vi "LUX_Intensity_test.vi"(8 "error in (no error)":errorcluster) -> (0 "error out":errorcluster)   [LabVIEW 2025]
uses:
  SubVIs/All test cluster.ctl
  SubVIs/All_enum_ctl.ctl
  SubVIs/Arduino_lamps.ctl
  SubVIs/Lamps_global.vi
  <vilib>/Utility/file.llb/Write Delimited Spreadsheet (string).vi
  <instrlib>/BK Precision 9200 Series/BK Precision 9200 Series.lvlib
  <instrlib>/Keithley 2260B/Keithley 2260B.lvlib
panel:
  in  "ESP PORT":refnum<visa-resource-name>
  out "Connected? 2":bool caption="Long Blank Button"
  in  "LUX VALUE":dbl
  out "Status":string
  in  "POWER SUPPLY":bool caption="Blank Button"
  out "Text name":string
  in  "COM PORT:":refnum<visa-resource-name>
  in  "Start/Stop":bool caption="Slide Switch"
  in  "File Path:":path
  in  "FILENAME":string
  out "Table":string[][](table)
  out "Connected?":bool caption="Long Blank Button"
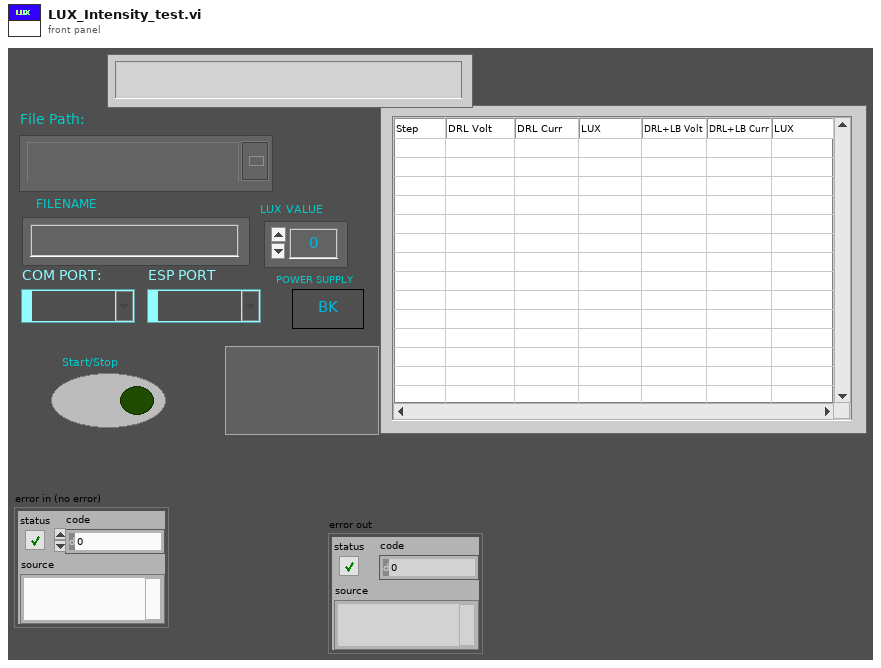
[diagram p1: front panel]
types:
  T1 = enum32{"Invalid", "Standard", "Closed", "Hidden", "Minimized", "Maximized"}
  T2 = typedef "All_enum_ctl.ctl" = enum16{"Init", "Poll", "Connect_esp32", "Connect", "check_start", "Start", "Set_Voltage", "On_relay", "Read_Voltage", "Off_Relay", "Next_Relay", "Next_Step", "Stop", "Store", "Error", "Exit"}
  T3 = typedef "All test cluster.ctl" = cluster{"FilePath":path, "Test Status":bool, "Start Volt":dbl, "End Volt":dbl, "Present Step":dbl, "Present Time(s)":dbl, "End Time":dbl, "Table":string[], "Intensity":string, "BK/Keith":bool, "COM":refnum<visa-resource-name>, "Next state":T2, "Step no.":dbl, "Start ms":u32, "ESP_COM":refnum<visa-resource-name>, "Relay_no":dbl, "Datas":string[]}
  T4 = typedef "Arduino_lamps.ctl" = enum16{"Init", "Poll", "Read", "Write", "Exit"}
  T5 = cluster{"Baud Rate":u32, "Parity":u16, "Data Bits":u16, "Stop Bits":u16, "Flow Control":u16}
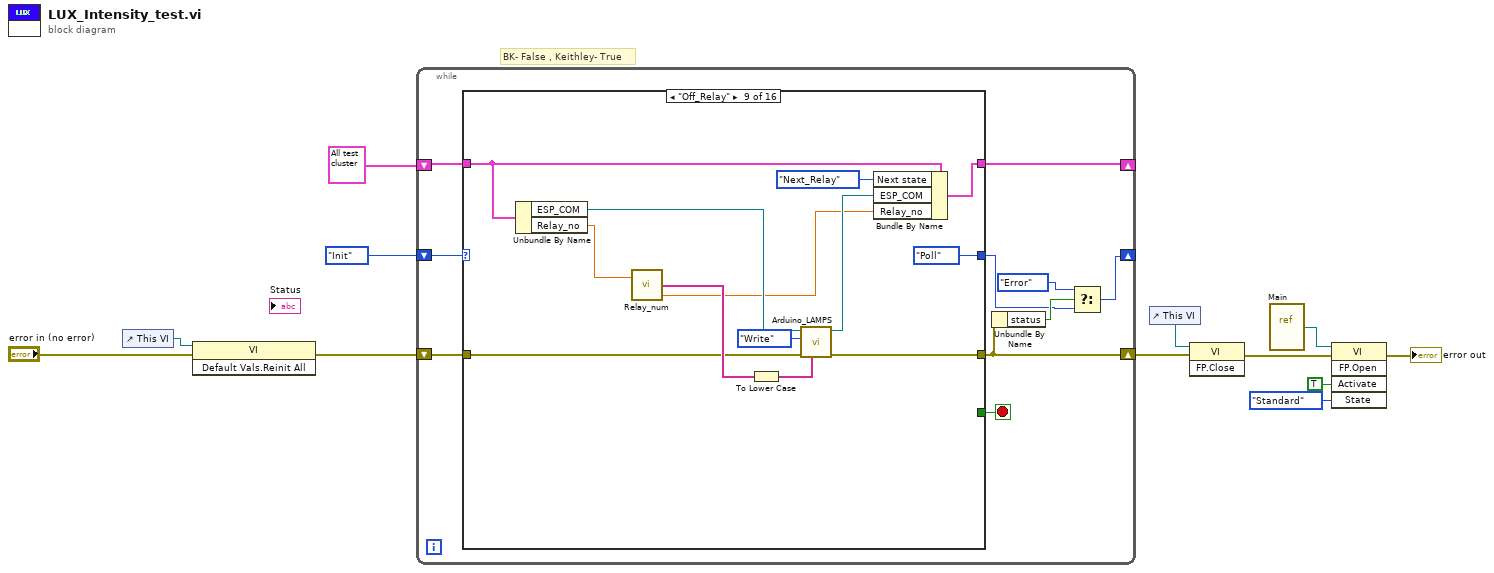
[diagram p0: block diagram]
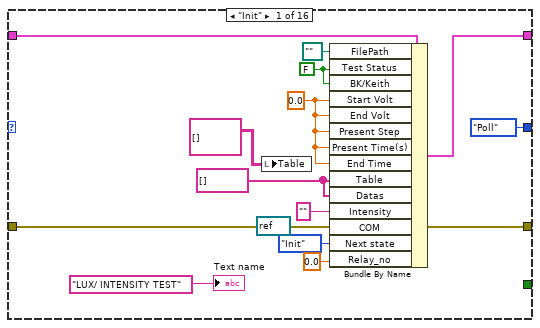
[diagram p2: hidden frame]
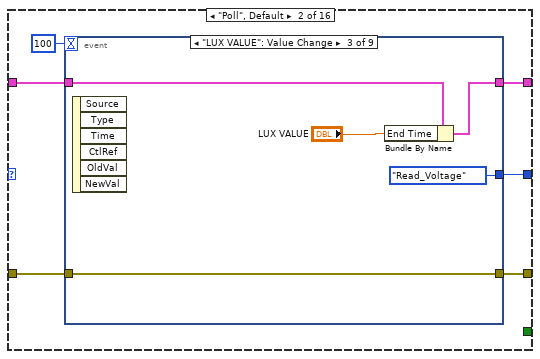
[diagram p3: hidden frame]
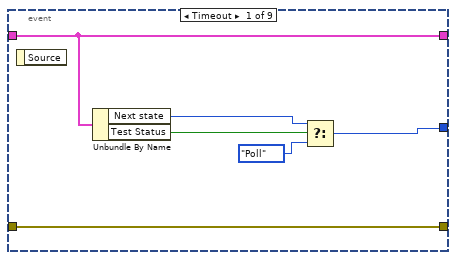
[diagram p4: hidden frame]
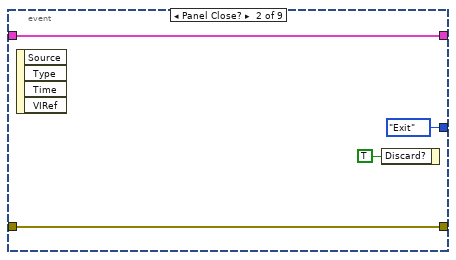
[diagram p5: hidden frame]
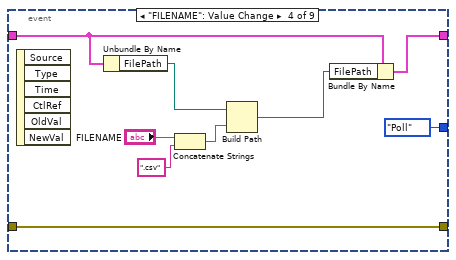
[diagram p6: hidden frame]
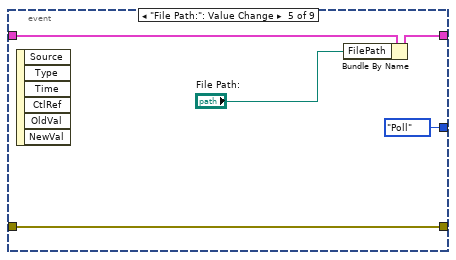
[diagram p7: hidden frame]
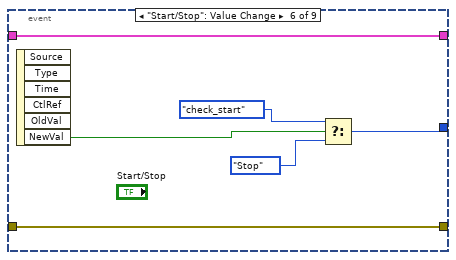
[diagram p8: hidden frame]
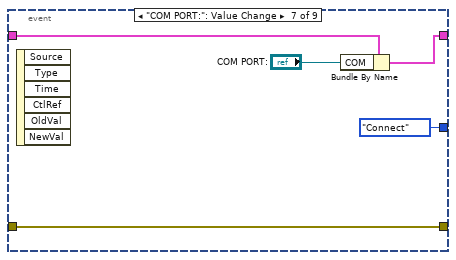
[diagram p9: hidden frame]
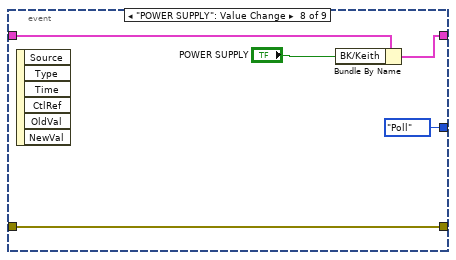
[diagram p10: hidden frame]
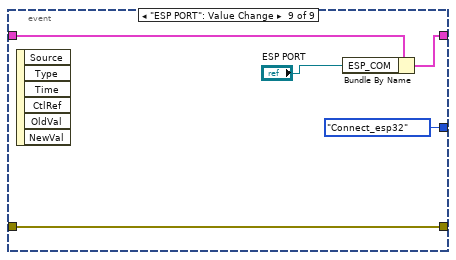
[diagram p11: hidden frame]
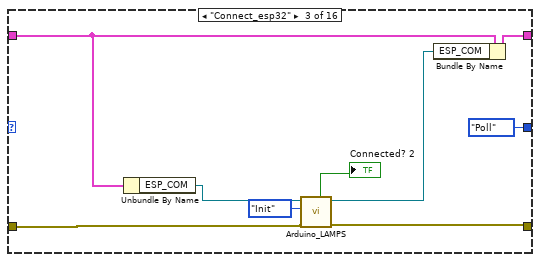
[diagram p12: hidden frame]
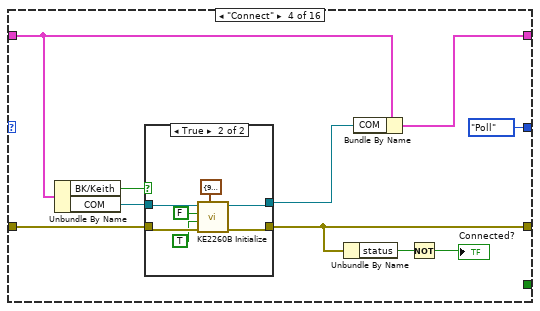
[diagram p13: hidden frame]
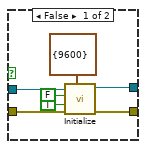
[diagram p14: hidden frame]
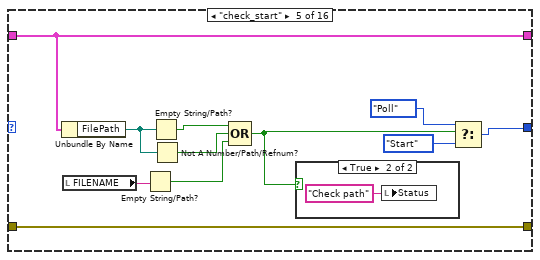
[diagram p15: hidden frame]
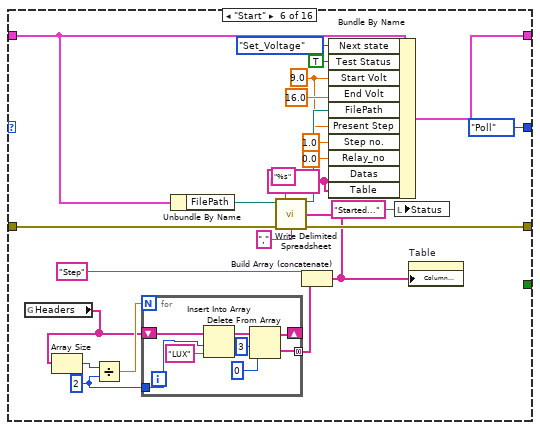
[diagram p17: hidden frame]
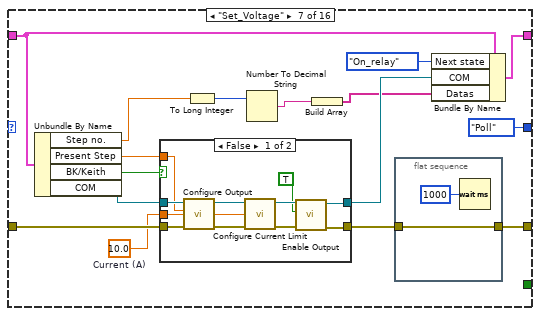
[diagram p18: hidden frame]
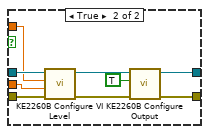
[diagram p19: hidden frame]
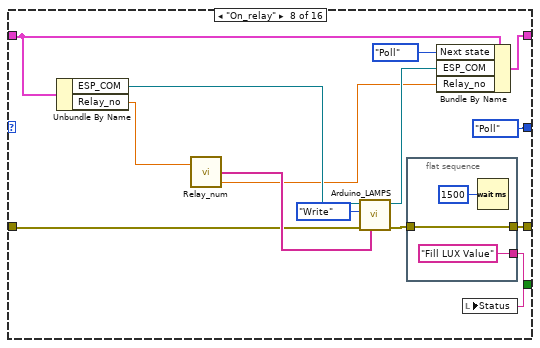
[diagram p20: hidden frame]
diagram:
  # "BK- False , Keithley- True"
  n1 = control-ref of="This VI"() -> (w12:refnum<vi>)
  n2 = invoke class="VI" method="Default Vals.Reinit All"(reference=w12, error in="error in (no error)") -> (error out=w10:errorcluster)  [unwired: 1 in, 2 out]
  n3 = while {
    shift-right: [w21] -> _
    shift-left: T3 {"FilePath"=path "", "Test Status"=FALSE, "Start Volt"=0.0, "End Volt"=0.0, "Present Step"=0.0, "Present Time(s)"=0.0, "End Time"=0.0, "Table"=[], "Intensity"="", "BK/Keith"=FALSE, "COM"="", "Next state"=enum."Init", "Step no."=0.0, "Start ms"=0, "ESP_COM"="", "Relay_no"=0.0, "Datas"=[]} -> [w20]
    shift-right: [w17] -> w2
    shift-left: w10 -> [w19]
    shift-right: [w13] -> _
    shift-left: All_enum_ctl."Init" -> [w22]
    stop <- w18 stop-if-true
    n4 = case shown="\"Off_Relay\"" w22 {
      tunnel: [w34 w39 w96 w103 w135 w160 w184 w209 w228 w251 w272 w303 w317 w332 w349 w369] -> w21
      tunnel: w20 -> [w36 w40 w97 w107 w135 w154 w183 w213 w229 w254 w273 w306 w311 w333 w352 w369]
      tunnel: w19 -> [w35 w42 w99 w111 w136 w156 w185 w212 w230 w255 w278 w307 w313 w337 w356 w374]
      tunnel: [w35 w41 w98 w106 w136 w155 w174 w211 w226 w241 w278 w300 w312 w337 w354 w370] -> w17
      tunnel: [All_enum_ctl."Poll" w37 All_enum_ctl."Poll" All_enum_ctl."Poll" w127 All_enum_ctl."Poll" All_enum_ctl."Poll" All_enum_ctl."Poll" All_enum_ctl."Poll" All_enum_ctl."Poll" All_enum_ctl."Poll" All_enum_ctl."Poll" All_enum_ctl."Poll" All_enum_ctl."Poll" All_enum_ctl."Poll" All_enum_ctl."Exit"] -> w14
      tunnel: [_ _ _ _ _ _ _ _ _ _ _ _ _ _ _ TRUE] -> w18
      frame "Init" {
        w25 = string[] [] ("Table")
        w32 = 0.0 ("Start Volt")
        w30 = FALSE ("Test Status")
        n5 = local write "Table"(string[][] [] ("Table")) -> ()
        n6 = Bundle By Name(cluster=w36, "FilePath"=path "", "Test Status"=w30, "BK/Keith"=w30, "Start Volt"=w32, "End Volt"=w32, "Present Step"=w32, "Present Time(s)"=w32, "End Time"=w32, "Table"=w25, "Datas"=w25, "Intensity"="", "COM"=refnum<visa-resource-name> refnum, "Next state"=All_enum_ctl."Init" ("Last state"), "Relay_no"=0.0) -> (w34:T3)
        "Text name" <- "LUX/ INTENSITY TEST"
      }
      frame "Poll", Default {
        n7 = event shown="[2] \"LUX VALUE\": Value Change" {
          selector: _ -> [_ _ _ _ _ _ _ _ _]
          dyn-events: _ -> [_ _ _ _ _ _ _ _ _]
          timeout: 100 -> [_ _ _ _ _ _ _ _ _]
          tunnel: w42 -> [w48 w49 w56 w66 w69 w72 w78 w83 w88]
          tunnel: [w48 w49 w56 w66 w69 w72 w78 w83 w88] -> w41
          tunnel: w40 -> [w47 w50 w57 w64 w71 w76 w82 w87 w92]
          tunnel: [w47 w50 w55 w60 w68 w76 w81 w86 w91] -> w39
          tunnel: [w44 All_enum_ctl."Exit" ("f") All_enum_ctl."Read_Voltage" ("f") All_enum_ctl."Poll" All_enum_ctl."Poll" w73 All_enum_ctl."Connect" ("f") All_enum_ctl."Poll" ("f") All_enum_ctl."Connect_esp32" ("f")] -> w37
          event Timeout {
            n8 = event-data() -> ()  [unwired: 1 in, 1 out]
            n9 = Unbundle By Name(w47) -> ("Next state"=w45:T2, "Test Status"=w43:bool)
            n10 = Select(t=w45, s=w43, f=All_enum_ctl."Poll") -> (s? t:f=w44:T2)
          }
          event Panel Close? {
            n11 = event-data() -> ()  [unwired: 1 in, 4 out]
            n12 = event-data("Discard?"=TRUE) -> ()  [unwired: 1 in, 1 out]
          }
          event "LUX VALUE": Value Change {
            n13 = event-data() -> ()  [unwired: 1 in, 6 out]
            n14 = Bundle By Name(cluster=w57, "End Time"="LUX VALUE") -> (w55:T3)
          }
          event "FILENAME": Value Change {
            n15 = event-data() -> ()  [unwired: 1 in, 6 out]
            n16 = Unbundle By Name(w64) -> ("FilePath"=w63:path)
            n17 = Concatenate Strings("FILENAME", ".csv" ("string")) -> (w62:string)
            n18 = Build Path(base path=w63, name or relative path=w62) -> (appended path=w59:path)
            n19 = Bundle By Name(cluster=w64, "FilePath"=w59) -> (w60:T3)
          }
          event "File Path:": Value Change {
            n20 = event-data() -> ()  [unwired: 1 in, 6 out]
            n21 = Bundle By Name(cluster=w71, "FilePath"="File Path:") -> (w68:T3)
          }
          event "Start/Stop": Value Change {
            n22 = event-data() -> ("NewVal"=w77:bool)  [unwired: 1 in, 5 out]
            n23 = Select(t=All_enum_ctl."check_start", s=w77, f=All_enum_ctl."Stop") -> (s? t:f=w73:T2)
          }
          event "COM PORT:": Value Change {
            n24 = event-data() -> ()  [unwired: 1 in, 6 out]
            n25 = Bundle By Name(cluster=w82, "COM"="COM PORT:") -> (w81:T3)
          }
          event "POWER SUPPLY": Value Change {
            n26 = event-data() -> ()  [unwired: 1 in, 6 out]
            n27 = Bundle By Name(cluster=w87, "BK/Keith"="POWER SUPPLY") -> (w86:T3)
          }
          event "ESP PORT": Value Change {
            n28 = event-data() -> ()  [unwired: 1 in, 6 out]
            n29 = Bundle By Name(cluster=w92, "ESP_COM"="ESP PORT") -> (w91:T3)
          }
        }
      }
      frame "Connect_esp32" {
        n30 = Unbundle By Name(w97) -> ("ESP_COM"=w101:refnum<visa-resource-name>)
        n31 = call "Arduino_LAMPS.vi"("error out"=w99, "Enum"=Arduino_lamps."Init", "VISA resource name"=w101) -> ("error out 2"=w98:errorcluster, "VISA out"=w95:refnum<visa-resource-name>, "status"=→"Connected? 2":bool)  [unwired: 4 in, 2 out]
        n32 = Bundle By Name(cluster=w97, "ESP_COM"=w95) -> (w96:T3)
      }
      frame "Connect" {
        n33 = Unbundle By Name(w107) -> ("BK/Keith"=w105:bool, "COM"=w104:refnum<visa-resource-name>)
        n34 = case shown="True" w105 {
          tunnel: w111 -> [w118 w125]
          tunnel: [w117 w124] -> w106
          tunnel: w104 -> [w116 w123]
          tunnel: [w112 w121] -> w102
          frame False {
            n35 = call <instrlib>:"Initialize.vi"("Serial Configuration"=cluster{"Baud Rate":u32} {"Baud Rate"=9600}, "error in (no error)"=w118, "Reset (True)"=TRUE, "ID Query (True)"=FALSE, "VISA resource name"=w116) -> ("error out"=w117:errorcluster, "VISA resource name out"=w112:refnum<visa-resource-name>)  [unwired: 5 in]
          }
          frame True {
            n36 = call <instrlib>:"KE2260B Initialize.vi"("Serial Configuration"=T5 {"Baud Rate"=9600, "Parity"=0, "Data Bits"=8, "Stop Bits"=10, "Flow Control"=0}, "error in (no error)"=w125, "Reset (True)"=TRUE, "ID Query (True)"=FALSE, "VISA resource name"=w123) -> ("error out"=w124:errorcluster, "VISA resource name out"=w121:refnum<visa-resource-name>)  [unwired: 5 in]
          }
        }
        n37 = Unbundle By Name(w106) -> ("status"=w110:bool)
        n38 = Bundle By Name(cluster=w107, "COM"=w102) -> (w103:T3)
        n39 = Not(x=w110) -> (.not. x?=→"Connected?":bool)
      }
      frame "check_start" {
        n40 = Unbundle By Name(w135) -> ("FilePath"=w133:path)
        n41 = local read "FILENAME"() -> (w134:string)
        n42 = Empty String/Path?(string/path=w134) -> (empty?=w130:bool)
        n43 = Empty String/Path?(string/path=w133) -> (empty?=w132:bool)
        n44 = Not A Number/Path/Refnum?(number/path/refnum=w133) -> (NaN/Path/Refnum?=w131:bool)
        n45 = Compound Arithmetic op=OR(w132, w131, w130) -> (w126:bool)
        n46 = case shown="True" w126 {
          frame False {
          }
          frame True {
            n47 = local write "Status"("Check path") -> ()
          }
        }
        n48 = Select(t=All_enum_ctl."Poll", s=w126, f=All_enum_ctl."Start") -> (s? t:f=w127:T2)
      }
      frame "Start" {
        w141 = 2 ("y")
        w144 = string[] [] ("Datas")
        w149 = 9.0 ("Start Volt")
        n49 = global read "Lamps_global.vi" "Headers"() -> (w140:string[])
        n50 = Array Size(array=w140) -> (size(s)=w142:i32)
        n51 = Divide(x=w142, y=w141) -> (x/y=w143:dbl)
        n52 = for {
          N: w143 -> [_]
          shift-right: [w163] -> _
          shift-left: w140 -> [w169]
          tunnel: w141 -> [w167]
          tunnel: [w162] -> w139 mode=concatenating
          n53 = Insert Into Array(array=w169, index=w167, new element="LUX" ("new element/subarray")) -> (w166:string[])
          n54 = Delete From Array(array=w166, length=3, index=0) -> (deleted portion=w162:string[], array with subset deleted=w163:string[])
        }
        n55 = Unbundle By Name(w154) -> ("FilePath"=w153:path)
        n56 = Build Array (concatenate)("Step" ("String"), w139) -> (w138:string[])
        n57 = call-poly <vilib>:"Write Delimited Spreadsheet.vi"("file path (dialog if empty)"=w153, "format (%s)"="%s" ("format (%.3f)"), "1D data"=w138, "error in (no error)"=w156, "delimiter (\\t)"="," ("delimiter (\\t)")) -> ("new file path (Not A Path if cancelled)"=w150:path, "error out"=w155:errorcluster)  [unwired: 9 in]
        n58 = Bundle By Name(cluster=w154, "Next state"=All_enum_ctl."Set_Voltage" ("Last state"), "Test Status"=TRUE, "Start Volt"=w149, "End Volt"=16.0, "FilePath"=w150, "Present Step"=w149, "Step no."=1.0, "Relay_no"=0.0, "Datas"=w144, "Table"=w144) -> (w160:T3)
        n59 = local write "Status"("Started..." ("Status")) -> ()
        n60 = property on="Table" class="Tbl (strict)"("Column Headers[]"=w138) -> ()  [unwired: 2 in, 2 out]
      }
      frame "Set_Voltage" {
        w177 = 10.0  # Current (A)
        n61 = Unbundle By Name(w183) -> ("Step no."=w171:dbl, "Present Step"=w178:dbl, "BK/Keith"=w179:bool, "COM"=w182:refnum<visa-resource-name>)
        n62 = case shown="False" w179 {
          tunnel: w185 -> [w189 w205]
          tunnel: [w196 w204] -> w175
          tunnel: w182 -> [w194 w202]
          tunnel: [w195 w200] -> w181
          tunnel: w178 -> [w193 w198]
          tunnel: w177 -> [w187 w197]
          frame False {
            n63 = call <instrlib>:"Configure Output.vi"("error in (no error)"=w189, "Voltage Level (0.0 V)"=w193, "VISA resource name"=w194) -> ("error out"=w190:errorcluster, "VISA resource name out"=w188:refnum<visa-resource-name>)  [unwired: 7 in]
            n64 = call <instrlib>:"Configure Current Limit.vi"("error in (no error)"=w190, "Current Limit (0.0 A)"=w187, "VISA resource name"=w188) -> ("error out"=w192:errorcluster, "VISA resource name out"=w191:refnum<visa-resource-name>)  [unwired: 7 in]
            n65 = call <instrlib>:"Enable Output.vi"("error in (no error)"=w192, "Enable Output (F: False)"=TRUE, "VISA resource name"=w191) -> ("error out"=w196:errorcluster, "VISA resource name out"=w195:refnum<visa-resource-name>)  [unwired: 7 in]
          }
          frame True {
            n66 = call <instrlib>:"KE2260B Configure VI Level.vi"("error in (no error)"=w205, "Current Level (0.000 A)"=w197, "Voltage Level (0.000 V)"=w198, "VISA resource name"=w202) -> ("error out"=w203:errorcluster, "VISA resource name out"=w201:refnum<visa-resource-name>)  [unwired: 6 in]
            n67 = call <instrlib>:"KE2260B Configure Output.vi"("error in (no error)"=w203, "Enable Output (T: Enable)"=TRUE, "VISA resource name"=w201) -> ("error out"=w204:errorcluster, "VISA resource name out"=w200:refnum<visa-resource-name>)  [unwired: 7 in]
          }
        }
        n68 = To Long Integer(number=w171) -> (32bit integer=w173:i32)
        n69 = Number To Decimal String(number=w173) -> (decimal integer string=w172:string)  [unwired: 1 in]
        n70 = Build Array(w172) -> (w170:string[])
        n71 = flat-sequence {
          tunnel: w175 -> [w207]
          tunnel: [w207] -> w174
          frame #0 {
            n72 = Wait (ms)(milliseconds to wait=u32 1000) -> ()  [unwired: 1 out]
          }
        }
        n73 = Bundle By Name(cluster=w183, "Next state"=All_enum_ctl."On_relay", "COM"=w181, "Datas"=w170) -> (w184:T3)
      }
      frame "On_relay" {
        n74 = Unbundle By Name(w213) -> ("ESP_COM"=w221:refnum<visa-resource-name>, "Relay_no"=w216:dbl)
        n75 = call "Relay_num.vi"("Relay_no."=w216) -> ("Relay"=w215:string[], "Relay_no.out"=w214:dbl)  [unwired: 1 in, 1 out]
        n76 = call "Arduino_LAMPS.vi"("DO's"=w215, "error out"=w212, "Enum"=Arduino_lamps."Write", "VISA resource name"=w221) -> ("error out 2"=w217:errorcluster, "VISA out"=w219:refnum<visa-resource-name>)  [unwired: 3 in, 3 out]
        n77 = flat-sequence {
          tunnel: w217 -> [w224]
          tunnel: [w224] -> w211
          tunnel: ["Fill LUX Value"] -> w208
          frame #0 {
            n78 = Wait (ms)(milliseconds to wait=u32 1500) -> ()  [unwired: 1 out]
          }
        }
        n79 = Bundle By Name(cluster=w213, "Next state"=All_enum_ctl."Poll", "ESP_COM"=w219, "Relay_no"=w214) -> (w209:T3)
        n80 = local write "Status"(w208) -> ()
      }
      frame "Off_Relay" {
        n81 = Unbundle By Name(w229) -> ("ESP_COM"=w237:refnum<visa-resource-name>, "Relay_no"=w233:dbl)
        n82 = call "Relay_num.vi"("Relay_no."=w233) -> ("Relay"=w232:string[], "Relay_no.out"=w231:dbl)  [unwired: 1 in, 1 out]
        n83 = To Lower Case(string=w232) -> (all lower case string=w225:string[])
        n84 = call "Arduino_LAMPS.vi"("DO's"=w225, "error out"=w230, "Enum"=Arduino_lamps."Write", "VISA resource name"=w237) -> ("error out 2"=w226:errorcluster, "VISA out"=w235:refnum<visa-resource-name>)  [unwired: 3 in, 3 out]
        n85 = Bundle By Name(cluster=w229, "Next state"=All_enum_ctl."Next_Relay", "ESP_COM"=w235, "Relay_no"=w231) -> (w228:T3)
      }
      frame "Read_Voltage" {
        n86 = Unbundle By Name(w254) -> ("Datas"=w238:string[], "BK/Keith"=w252:bool, "COM"=w253:refnum<visa-resource-name>, "End Time"=w243:dbl)
        n87 = case shown="False" w252 {
          tunnel: w255 -> [w261 w267]
          tunnel: [w260 w266] -> w242
          tunnel: w253 -> [w259 w264]
          tunnel: [w258 w265] -> w250
          tunnel: [w257 w263] -> w247
          tunnel: [w256 w262] -> w246
          frame False {
            n88 = call <instrlib>:"Read Output.vi"("VISA resource name"=w259, "error in (no error)"=w261) -> ("VISA resource name out"=w258:refnum<visa-resource-name>, "Actual Voltage Level (V)"=w257:dbl, "Actual Current Level (A)"=w256:dbl, "error out"=w260:errorcluster)  [unwired: 9 in, 1 out]
          }
          frame True {
            n89 = call <instrlib>:"KE2260B Read Output.vi"("error in (no error)"=w267, "VISA resource name"=w264) -> ("error out"=w266:errorcluster, "Actual Current Level (A)"=w262:dbl, "Actual Voltage Level (V)"=w263:dbl, "VISA resource name out"=w265:refnum<visa-resource-name>)  [unwired: 6 in]
          }
        }
        n90 = Build Array(w247, w246, w243) -> (w245:dbl[])
        n91 = for {
          tunnel: w245 -> [w269] mode=indexing
          tunnel: [w268] -> w244 mode=indexing
          n92 = Number To Fractional String(number=w269, precision (6)=i16 2) -> (F-format string=w268:string)  [unwired: 2 in]
        }
        n93 = Build Array (concatenate)(w238, w244) -> (w239:string[])
        n94 = Bundle By Name(cluster=w254, "Next state"=All_enum_ctl."Off_Relay", "COM"=w250, "Datas"=w239) -> (w251:T3)
        n95 = property on="Status" class="Str"(error in=w242, "Value"="" ("Status")) -> (error out=w241:errorcluster)  [unwired: 1 in, 1 out]
      }
      frame "Next_Relay" {
        n96 = Unbundle By Name(w273) -> ("Relay_no"=w277:dbl, "Datas"=w274:string[])
        n97 = call "Relay_num.vi"("Relay_no."=w277) -> ("x = y?"=w276:bool, "Relay_no.out"=w275:dbl)  [unwired: 1 in, 1 out]
        n98 = case shown="False" w276 {
          tunnel: [w288 w293] -> w272
          tunnel: w273 -> [w287 w292]
          tunnel: w275 -> [w285 _]
          tunnel: w274 -> [w279 w289]
          frame False {
            n99 = local read "Table"() -> (w283:string[][])
            n100 = Increment(x=w285) -> (x+1=w284:dbl)
            n101 = Array Size(array=w283) -> (size(s)=w281:i32[])
            n102 = Index Array(array=w281) -> (element=w280:i32)  [unwired: 1 in]
            n103 = Bundle By Name(cluster=w287, "Next state"=All_enum_ctl."On_relay", "Relay_no"=w284, "Datas"=w279) -> (w288:T3)
            n104 = Replace Array Subset(array=w283, new element=w279, index (row)=w280) -> (w282:string[][])  [unwired: 1 in]
            n105 = local write "Table"(w282) -> ()
          }
          frame True {
            n106 = Bundle By Name(cluster=w292, "Next state"=All_enum_ctl."Store", "Relay_no"=0.0, "Table"=w289) -> (w293:T3)
          }
        }
      }
      frame "Store" {
        n107 = Unbundle By Name(w306) -> ("Table"=w297:string[], "FilePath"=w299:path)
        n108 = local read "Table"() -> (w305:string[][])
        n109 = Build Array (concatenate)(w305, w297) -> (→"Table":string[][])
        n110 = call-poly <vilib>:"Write Delimited Spreadsheet.vi"("file path (dialog if empty)"=w299, "format (%s)"="%s", "1D data"=w297, "append to file? (new file:F)"=TRUE, "error in (no error)"=w307, "delimiter (\\t)"="," ("delimiter (\\t)")) -> ("new file path (Not A Path if cancelled)"=w296:path, "error out"=w300:errorcluster)  [unwired: 8 in]
        n111 = Bundle By Name(cluster=w306, "Next state"=All_enum_ctl."Next_Step", "FilePath"=w296) -> (w303:T3)
      }
      frame "Stop" {
        n112 = Unbundle By Name(w311) -> ("BK/Keith"=w314:bool, "COM"=w315:refnum<visa-resource-name>)
        n113 = case shown="False" w314 {
          tunnel: [w323 w327] -> w312
          tunnel: w315 -> [w321 w326]
          tunnel: [w322 w325] -> w310
          tunnel: w313 -> [w319 _]
          frame False {
            n114 = call <instrlib>:"Enable Output.vi"("error in (no error)"=w319, "Enable Output (F: False)"=FALSE, "VISA resource name"=w321) -> ("error out"=w323:errorcluster, "VISA resource name out"=w322:refnum<visa-resource-name>)  [unwired: 7 in]
          }
          frame True {
            n115 = call <instrlib>:"KE2260B Configure Output.vi"("Enable Output (T: Enable)"=FALSE, "VISA resource name"=w326) -> ("error out"=w327:errorcluster, "VISA resource name out"=w325:refnum<visa-resource-name>)  [unwired: 8 in]
          }
        }
        n116 = local write "Start/Stop"(FALSE ("Start/Stop")) -> ()
        n117 = local write "Status"("Test Stopped...." ("Status")) -> ()
        n118 = Bundle By Name(cluster=w311, "Test Status"=FALSE, "COM"=w310) -> (w317:T3)
      }
      frame "Next_Step" {
        n119 = Unbundle By Name(w333) -> ("Present Step"=w334:dbl, "End Volt"=w335:dbl, "Step no."=w330:dbl)
        n120 = Greater Or Equal?(x=w334, y=w335) -> (x >= y?=w336:bool)
        n121 = case shown="False" w336 {
          tunnel: w334 -> [_ _]
          tunnel: w333 -> [w344 w347]
          tunnel: [w343 w346] -> w332
          tunnel: w330 -> [w341 _]
          tunnel: dbl[] [0.0, 9.0, 12.0, 16.0] -> [w340 _]
          frame False {
            n122 = Increment(x=w341) -> (x+1=w339:dbl)
            n123 = Index Array(array=w340, index=w339) -> (element=w338:dbl)
            n124 = Bundle By Name(cluster=w344, "Next state"=All_enum_ctl."Set_Voltage", "Present Step"=w338, "Step no."=w339) -> (w343:T3)
          }
          frame True {
            n125 = Bundle By Name(cluster=w347, "Next state"=All_enum_ctl."Stop") -> (w346:T3)
          }
        }
        n126 = local write "LUX VALUE"(0.0 ("LUX VALUE")) -> ()
      }
      frame "Error" {
        n127 = Unbundle By Name(w352) -> ("BK/Keith"=w350:bool, "COM"=w351:refnum<visa-resource-name>)
        n128 = case shown="False" w350 {
          tunnel: w356 -> [w359 w364]
          tunnel: [w360 w363] -> w353
          tunnel: w351 -> [w358 w362]
          tunnel: [w357 w361] -> w348
          frame False {
            n129 = call <instrlib>:"Reset.vi"("error in (no error)"=w359, "VISA resource name"=w358) -> ("error out"=w360:errorcluster, "VISA resource name out"=w357:refnum<visa-resource-name>)  [unwired: 8 in]
          }
          frame True {
            n130 = call <instrlib>:"KE2260B Reset.vi"("error in (no error)"=w364, "VISA resource name"=w362) -> ("error out"=w363:errorcluster, "VISA resource name out"=w361:refnum<visa-resource-name>)  [unwired: 8 in]
          }
        }
        n131 = call <vilib>:"Clear Errors.vi"("error in (no error)"=w353) -> ("error out"=w354:errorcluster)  [unwired: 5 in, 1 out]
        n132 = Bundle By Name(cluster=w352, "COM"=w348) -> (w349:T3)
      }
      frame "Exit" {
        n133 = Unbundle By Name(w369) -> ("ESP_COM"=w365:refnum<visa-resource-name>, "BK/Keith"=w367:bool, "COM"=w368:refnum<visa-resource-name>)
        n134 = case shown="False" w367 {
          tunnel: w374 -> [w377 w380]
          tunnel: [w376 w379] -> w371
          tunnel: w368 -> [w375 w378]
          frame False {
            n135 = call <instrlib>:"Close.vi"("error in (no error)"=w377, "VISA resource name"=w375) -> ("error out"=w376:errorcluster)  [unwired: 9 in]
          }
          frame True {
            n136 = call <instrlib>:"KE2260B Close.vi"("error in (no error)"=w380, "VISA resource name"=w378) -> ("error out"=w379:errorcluster)  [unwired: 9 in]
          }
        }
        n137 = VISA Close(VISA resource name=w365, error in (no error)=w371) -> (error out=w366:errorcluster)
        n138 = call <vilib>:"Clear Errors.vi"("error in (no error)"=w366) -> ("error out"=w370:errorcluster)  [unwired: 5 in, 1 out]
      }
    }
    n139 = Unbundle By Name(w17) -> ("status"=w16:bool)
    n140 = Select(t=All_enum_ctl."Error", s=w16, f=w14) -> (s? t:f=w13:T2)
  }
  n141 = control-ref of="This VI"() -> (w3:refnum<vi>)
  n142 = invoke class="VI" method="FP.Close"(reference=w3, error in=w2) -> (error out=w1:errorcluster)  [unwired: 1 in, 2 out]
  n143 = vi-ref "Main.vi"() -> (w7:refnum<vi>)
  n144 = invoke class="VI" method="FP.Open"(reference=w7, error in=w1, "Activate"=TRUE ("Activate?"), "State"=T1."Standard") -> (error out=→"error out":errorcluster)  [unwired: 1 in, 4 out]
